vi "Open Template.vi"() -> ()   [LabVIEW 2021]
doc: "::: CalcExpress Toolkit :::\nCopyright (c) 2000-2026 Konstantin Shifershteyn. All rights reserved."
uses:
  vi.lib/addons/CalcExpress/cemisc.llb/[ce] CE component paths - Kind of Path Enum.ctl
  <vilib>/event_ctls.llb/eventvkey.ctl
panel:
  out "Icon":picture
  in  "Open":bool
  out "description":string
  in  "Exit":bool
  in  "VI List":i32(listbox) caption="Templates (double click a list item to open the template)"
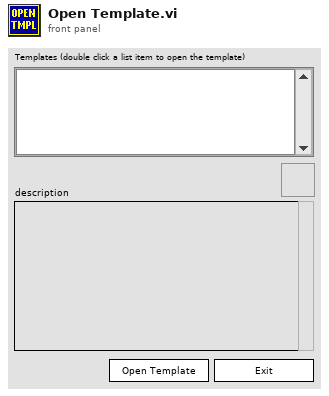
[diagram p1: front panel]
types:
  T1 = typedef "[ce] CE component paths - Kind of Path Enum.ctl" = enum16{"VIs", "FuncVIs", "Help", "Examples", "Project", "Templates"}
  T2 = typedef "eventvkey.ctl" = enum16{"ASCII", "Enter", "Return", "Shift", "Ctrl", "Alt", "Cmd", "Opt", "Caps", "NumLock", "Clear", "Break", "Up", "Down", "Left", "Right", "Insert", "Delete", "Home", "End", "PageUp", "PageDown", "Escape", "Help", "Pause", "ScrollLock", "F1", "F2", "F3", "F4", "F5", "F6", "F7", "F8", "F9", "F10", "F11", "F12", "F13", "F14", "F15", "F16", "F17", "F18", "F19", "F20", "F21", "F22", "F23", "F24", "Play", "VolumeUp", "VolumeDown", "Mute", "Two Byte Char"}
  T3 = typedef "imagedata.ctl" = cluster{"image type":i32, "image depth":i32, "image":u8[], "mask":u8[], "colors":u32[], "Rectangle":cluster{"left":i16, "top":i16, "right":i16, "bottom":i16}}
  T4 = cluster{"Shift":bool, "Ctrl":bool, "Alt":bool, "Cmd":bool, "Opt":bool}
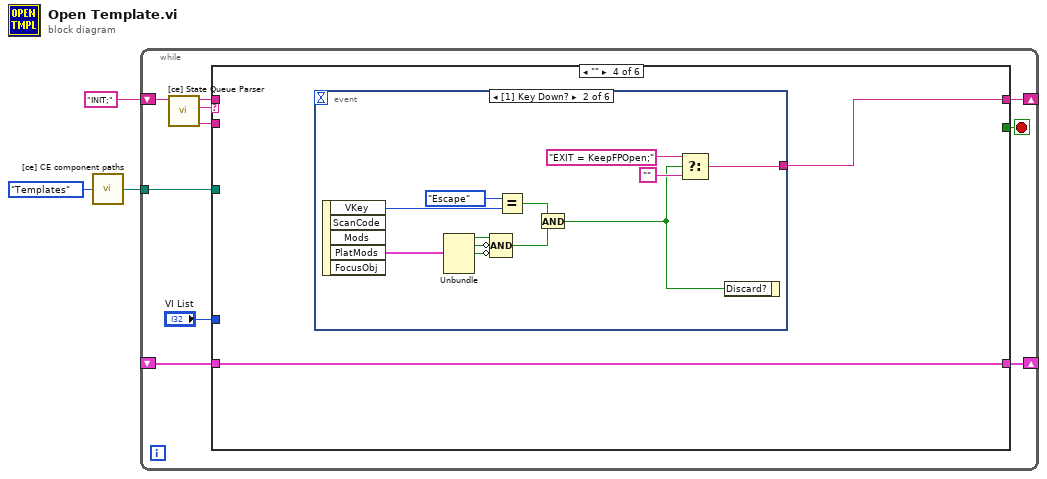
[diagram p0: block diagram]
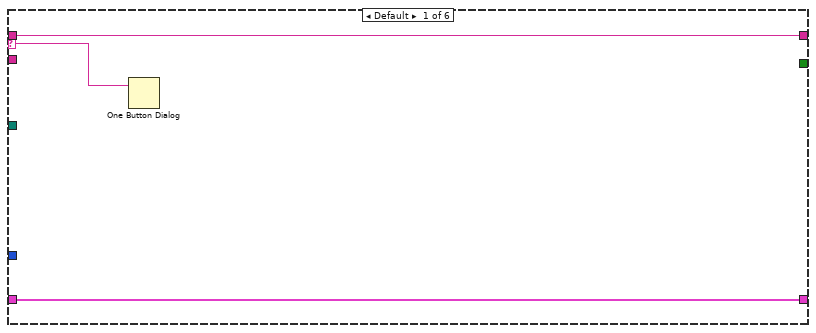
[diagram p2: hidden frame]
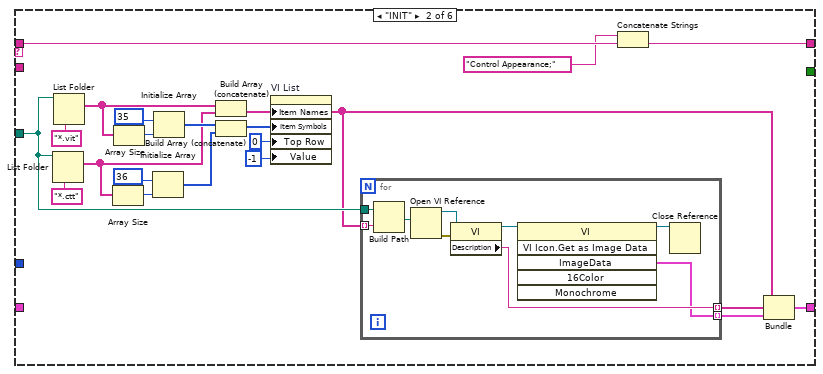
[diagram p3: hidden frame]
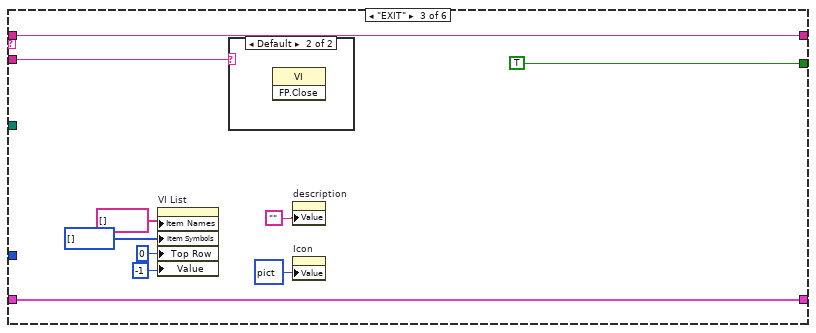
[diagram p4: hidden frame]
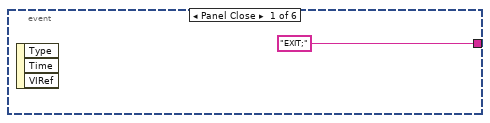
[diagram p6: hidden frame]
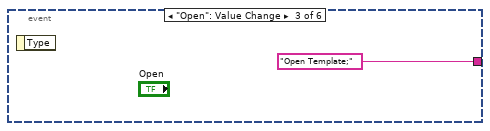
[diagram p7: hidden frame]
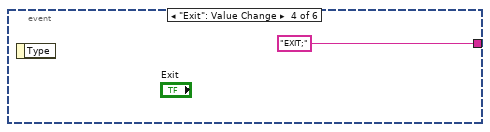
[diagram p8: hidden frame]
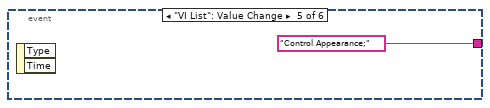
[diagram p9: hidden frame]
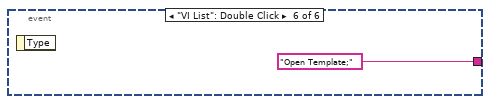
[diagram p10: hidden frame]
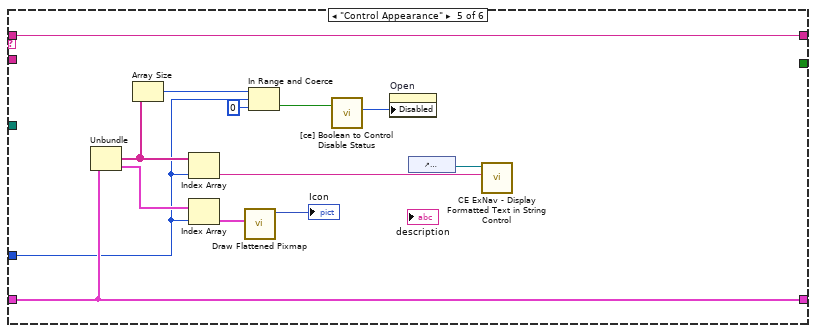
[diagram p11: hidden frame]
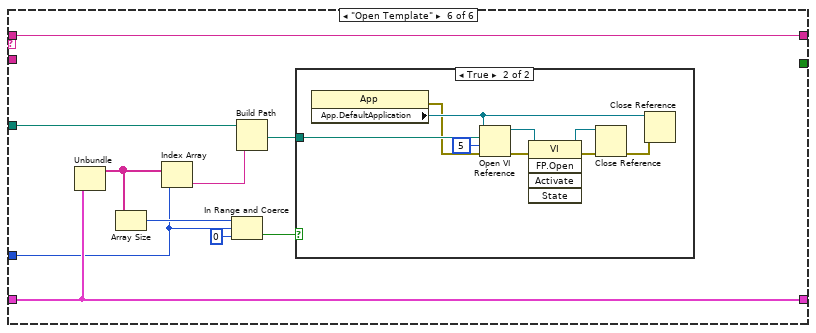
[diagram p12: hidden frame]
diagram:
  n1 = call "[ce] CE component paths.vi"("kind of path"=[ce]_CE_component_paths_-_Kind_of_Path_Enum."Templates") -> ("path out"=w1:path)  [unwired: 1 in]
  n2 = while {
    shift-right: [w11] -> _
    shift-left: "INIT;" -> [w13]
    tunnel: w1 -> [w8]
    shift-right: [w7] -> _
    shift-left: _ -> [w6]
    stop <- w9 stop-if-true
    n3 = call "[ce] State Queue Parser.vi"("input queue"=w13) -> ("state parameters"=w4:string, "state"=w12:string, "remained queue"=w10:string)  [unwired: 6 in]
    n4 = case shown="\"\"" w12 {
      selector: w12 -> [w16 _ _ _ _ _]
      tunnel: [w15 w23 w55 w57 w88 w98] -> w11
      tunnel: w10 -> [w15 w24 w55 _ w88 w98]
      tunnel: [_ _ TRUE _ _ _] -> w9
      tunnel: w8 -> [_ w22 _ _ _ w95]
      tunnel: [w14 w20 w50 w58 w87 w97] -> w7
      tunnel: w6 -> [w14 _ w50 w58 w87 w97]
      tunnel: "VI List" -> [_ _ _ _ w80 w90]
      tunnel: w4 -> [_ _ w47 _ _ _]
      frame Default {
        n5 = One Button Dialog(message=w16) -> ()  [unwired: 1 in, 1 out]
      }
      frame "INIT" {
        n6 = List Folder(path=w22, pattern="*.ctt") -> (filenames=w32:string[])  [unwired: 2 in, 3 out]
        n7 = List Folder(path=w22, pattern="*.vit") -> (filenames=w31:string[])  [unwired: 2 in, 3 out]
        n8 = Array Size(array=w32) -> (size(s)=w30:i32)
        n9 = Array Size(array=w31) -> (size(s)=w27:i32)
        n10 = Initialize Array(36, w30) -> (w34:i32[])
        n11 = Initialize Array(35, w27) -> (w33:i32[])
        n12 = Build Array (concatenate)(w31, w32) -> (w21:string[])
        n13 = Build Array (concatenate)(w33, w34) -> (w36:i32[])
        n14 = property on="VI List" class="LstBox (strict)"("Item Names"=w21, "Item Symbols"=w36, "Top Row"=0, "Value"=-1 ("list")) -> ()  [unwired: 2 in, 2 out]
        n15 = for {
          tunnel: w21 -> [w44] mode=indexing
          tunnel: w22 -> [w43]
          tunnel: [w39] -> w18 mode=indexing
          tunnel: [w38] -> w17 mode=indexing
          n16 = Build Path(base path=w43, name or relative path=w44) -> (appended path=w46:path)
          n17 = Open VI Reference(vi path=w46) -> (vi reference=w42:refnum<vi>, error out=w45:errorcluster)  [unwired: 5 in]
          n18 = property class="VI"(reference=w42, error in=w45) -> (reference out=w41:refnum<vi>, "Description"=w39:string)  [unwired: 1 out]
          n19 = invoke class="VI" method="VI Icon.Get as Image Data"(reference=w41) -> (reference out=w40:refnum<vi>, "ImageData"=w38:T3)  [unwired: 5 in, 4 out]
          n20 = Close Reference(reference=w40) -> ()  [unwired: 1 in, 1 out]
        }
        n21 = Concatenate Strings("Control Appearance;" ("string"), w24) -> (w23:string)
        n22 = Bundle(w21, w18, w17) -> (w20:cluster{string[], string[], T3[]})  [unwired: 1 in]
      }
      frame "EXIT" {
        n23 = property on="VI List" class="LstBox (strict)"("Item Names"=string[] [], "Item Symbols"=i32[] [], "Top Row"=0, "Value"=-1 ("list")) -> ()  [unwired: 2 in, 2 out]
        n24 = case shown="Default" w47 {
          frame "KeepFPOpen" {
          }
          frame Default {
            n25 = invoke class="VI" method="FP.Close"() -> ()  [unwired: 3 in, 3 out]
          }
        }
        n26 = property on="description" class="Str"("Value"="") -> ()  [unwired: 2 in, 2 out]
        n27 = property on="Icon" class="Pict"("Value"=picture data[5B] ("Icon")) -> ()  [unwired: 2 in, 2 out]
      }
      frame "" {
        n28 = event shown="[1] Key Down?" {
          selector: _ -> [_ _ _ _ _ _]
          dyn-events: _ -> [_ _ _ _ _ _]
          timeout: _ -> [_ _ _ _ _ _]
          tunnel: ["EXIT;" w61 "Open Template;" "EXIT;" "Control Appearance;" "Open Template;"] -> w57
          event Panel Close {
            n29 = event-data() -> ()  [unwired: 1 in, 3 out]
          }
          event Key Down? {
            n30 = event-data() -> ("VKey"=w65:T2, "PlatMods"=w64:T4)  [unwired: 1 in, 3 out]
            n31 = Unbundle(w64) -> ("Shift"=w70:bool, "Ctrl"=w69:bool, "Alt"=w68:bool)  [unwired: 2 out]
            n32 = Compound Arithmetic op=AND(w70, invert w69, invert w68) -> (w67:bool)
            n33 = Equal?(x=eventvkey."Escape", y=w65) -> (x = y?=w66:bool)
            n34 = And(x=w66, y=w67) -> (x .and. y?=w60:bool)
            n35 = Select(t="EXIT = KeepFPOpen;", s=w60, f="") -> (s? t:f=w61:string)
            n36 = event-data("Discard?"=w60) -> ()  [unwired: 1 in, 1 out]
          }
          event "Open": Value Change {
            n37 = event-data() -> ()  [unwired: 1 in, 1 out]
          }
          event "Exit": Value Change {
            n38 = event-data() -> ()  [unwired: 1 in, 1 out]
          }
          event "VI List": Value Change {
            n39 = event-data() -> ()  [unwired: 1 in, 2 out]
          }
          event "VI List": Double Click {
            n40 = event-data() -> ()  [unwired: 1 in, 1 out]
          }
        }
      }
      frame "Control Appearance" {
        n41 = Unbundle(w87) -> (w84:string[], w81:T3[])  [unwired: 1 out]
        n42 = Array Size(array=w84) -> (size(s)=w85:i32)
        n43 = Index Array(array=w84, index=w80) -> (element=w77:string)
        n44 = Index Array(array=w81, index=w80) -> (element=w79:T3)
        n45 = call <vilib>:"Draw Flattened Pixmap.vi"("image data"=w79) -> ("new picture"=→"Icon":picture)  [unwired: 8 in]
        n46 = In Range and Coerce(upper limit=w85, x=w80, lower limit=0) -> (In Range?=w83:bool)  [unwired: 1 out]
        n47 = call "[ce] Boolean to Control Disable Status.vi"("Status in"=w83) -> ("Control Disable if False"=w82:u8)  [unwired: 3 in, 1 out]
        n48 = property on="Open" class="Bool"("Disabled"=w82) -> ()  [unwired: 2 in, 2 out]
        n49 = control-ref of="description"() -> (w76:refnum<vi>)
        n50 = call "CE ExNav - Display Formatted Text in String Control.vi"("Formatted text"=w77, "Str Refnum"=w76) -> ()  [unwired: 8 in, 2 out]
      }
      frame "Open Template" {
        n51 = Unbundle(w97) -> (w91:string[])  [unwired: 2 out]
        n52 = Array Size(array=w91) -> (size(s)=w92:i32)
        n53 = Index Array(array=w91, index=w90) -> (element=w94:string)
        n54 = In Range and Coerce(upper limit=w92, x=w90, lower limit=0) -> (In Range?=w89:bool)  [unwired: 1 out]
        n55 = Build Path(base path=w95, name or relative path=w94) -> (appended path=w96:path)
        n56 = case shown="True" w89 {
          tunnel: w96 -> [_ w105]
          frame False {
          }
          frame True {
            n57 = property class="App"() -> (error out=w100:errorcluster, "App.DefaultApplication"=w102:refnum<vi>)  [unwired: 2 in, 1 out]
            n58 = Open VI Reference(application reference (local)=w102, vi path=w105, options=5, error in (no error)=w100) -> (vi reference=w106:refnum<vi>, error out=w104:errorcluster)  [unwired: 2 in]
            n59 = invoke class="VI" method="FP.Open"(reference=w106, error in=w104) -> (reference out=w107:refnum<vi>, error out=w103:errorcluster)  [unwired: 3 in, 3 out]
            n60 = Close Reference(reference=w107, error in (no error)=w103) -> (error out=w101:errorcluster)
            n61 = Close Reference(reference=w102, error in (no error)=w101) -> ()  [unwired: 1 out]
          }
        }
      }
    }
  }
